vi "Commentaire fichier acqui.vi"(11 "Chemin":path) -> (3 "Chaîne":string)   [LabVIEW 2022 SP3]
uses:
  Variables globales/Variable globale compteurs.vi
  Variables globales/Variable glob generale.vi
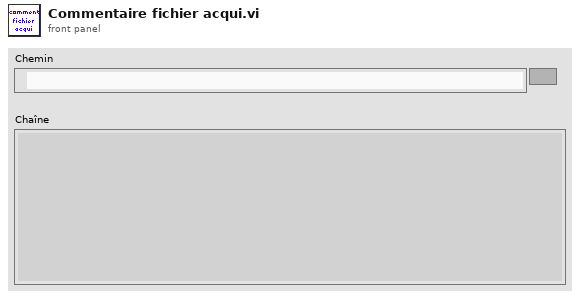
[diagram p1: front panel]
types:
  T1 = cluster{"Nom tache compteurs":refnum<k21>, "Noms des compteurs":string[], "Selection":bool[], "Init compteurs":dbl[], "Noms compteurs selectionnes":string[]}
  T2 = typedef "LVDateTimeRec.ctl" = cluster{"fraction de seconde":dbl, "seconde":i32, "minute":i32, "heure":i32, "jour du mois":i32, "mois":i32, "année":i32, "jour de la semaine":i32, "jour de l'année":i32, "DST":i32}
  T3 = enum16{"open", "replace", "create", "open or create", "replace or create", "replace or create with confirmation"}
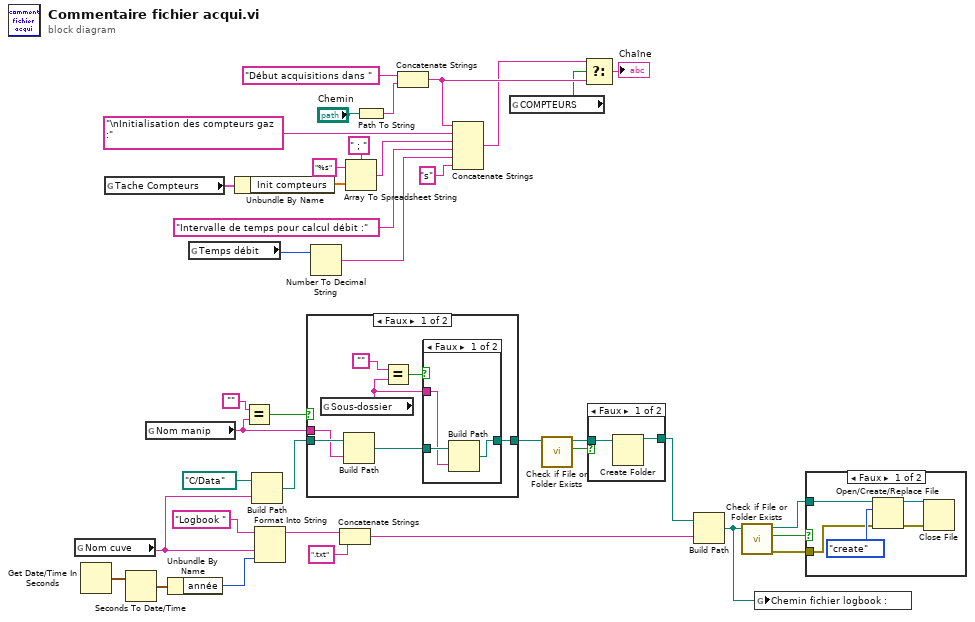
[diagram p0: block diagram]
diagram:
  n1 = global read "Variable glob generale.vi" "Nom cuve"() -> (w21:string)
  n2 = Get Date/Time In Seconds() -> (seconds since 1Jan1904=w11:timestamp)
  n3 = global read "Variable globale compteurs.vi" "Tache Compteurs"() -> (w31:T1)
  n4 = Seconds To Date/Time(time stamp (now)=w11) -> (date time rec=w12:T2)  [unwired: 1 in]
  n5 = global read "Variable glob generale.vi" "Nom manip"() -> (w7:string)
  n6 = Unbundle By Name(w12) -> ("année"=w17:i32)
  n7 = global read "Variable globale compteurs.vi" "Temps débit"() -> (w25:u16)
  n8 = Unbundle By Name(w31) -> ("Init compteurs"=w32:dbl[])
  n9 = Equal?(x="", y=w7) -> (x = y?=w10:bool)
  n10 = Build Path(base path=path "C:/Data", name or relative path=w21) -> (appended path=w9:path)
  n11 = Format Into String(initial string="Logbook ", w21, w17) -> (resulting string=w16:string)  [unwired: 2 in, 1 out]
  n12 = case shown="Faux" w10 {
    tunnel: w9 -> [w45 w50]
    tunnel: [w40 w50] -> w4
    tunnel: w7 -> [w44 _]
    frame False {
      n13 = global read "Variable glob generale.vi" "Sous-dossier"() -> (w39:string)
      n14 = Build Path(base path=w45, name or relative path=w44) -> (appended path=w41:path)
      n15 = Equal?(x="", y=w39) -> (x = y?=w42:bool)
      n16 = case shown="Faux" w42 {
        tunnel: w41 -> [w48 w49]
        tunnel: [w46 w49] -> w40
        tunnel: w39 -> [w47 _]
        frame False {
          n17 = Build Path(base path=w48, name or relative path=w47) -> (appended path=w46:path)
        }
        frame True {
        }
      }
    }
    frame True {
    }
  }
  n18 = Number To Decimal String(number=w25) -> (decimal integer string=w23:string)  [unwired: 1 in]
  n19 = Concatenate Strings(w16, ".txt") -> (w15:string)
  n20 = Array To Spreadsheet String(delimiter (Tab)=" ; " ("séparateur (Tabulation)"), array=w32, 3:"%s" ("chaîne de format")) -> (spreadsheet string=w36:string)
  n21 = Path To String(path="Chemin") -> (string=w27:string)
  n22 = Concatenate Strings("Début acquisitions dans ", w27) -> (w38:string)
  n23 = Concatenate Strings(w38, "\nInitialisation des compteurs gaz :", w36, "Intervalle de temps pour calcul débit :", w23, "s") -> (w37:string)
  n24 = global read "Variable globale compteurs.vi" "COMPTEURS"() -> (w29:bool)
  n25 = call <vilib>:"Check if File or Folder Exists.vi"("path"=w4) -> ("file or folder exists?"=w3:bool, "dup path"=w2:path)  [unwired: 8 in, 1 out]
  n26 = Select(t=w37, s=w29, f=w38) -> (s? t:f=→"Chaîne":string)
  n27 = case shown="Faux" w3 {
    tunnel: w2 -> [w52 w53]
    tunnel: [w51 w53] -> w1
    frame False {
      n28 = Create Folder(path (use dialog)=w52) -> (created path=w51:path)  [unwired: 2 in, 2 out]
    }
    frame True {
    }
  }
  n29 = Build Path(base path=w1, name or relative path=w15) -> (appended path=w14:path)
  n30 = call <vilib>:"Check if File or Folder Exists.vi"("path"=w14) -> ("error out"=w5:errorcluster, "file or folder exists?"=w13:bool, "dup path"=w6:path)  [unwired: 8 in]
  n31 = global write "Variable glob generale.vi" "Chemin fichier logbook :"(w14) -> ()
  n32 = case shown="Faux" w13 {
    tunnel: w6 -> [w57 _]
    tunnel: w5 -> [w54 _]
    frame False {
      n33 = Open/Create/Replace File(file path (use dialog)=w57, error in=w54, operation (0:open)=T3."create" ("opération (0 : open)")) -> (refnum out=w56:refnum<file>, error out=w55:errorcluster)  [unwired: 3 in, 1 out]
      n34 = Close File(refnum=w56, error in=w55) -> ()  [unwired: 2 out]
    }
    frame True {
    }
  }
